vi "OverlayBitmapCenter.vi"(7 "GroupName":string, 8 "error in":errorcluster, 9 "Bitmap":u32[][](array[colorbox]), 10 "Center":T1, 11 "Image Reference In":T2) -> (0 "error out":errorcluster, 3 "Image Reference Out":T2)   [LabVIEW 2020, in "OpenLvVision_Overlays.lvlib"]
doc: "Overlays an bitmap on top of an image."
uses:
  OpenLvVision_Overlays.lvlib
  <vilib>/OpenLvVision/OpenLvVision_Image/Management/TypeDef/OLV Image.ctl
  TypeDefs/PointI32.ctl
  <vilib>/OpenLvVision/OpenLvVision_Image/Management/OLV Management.lvlib
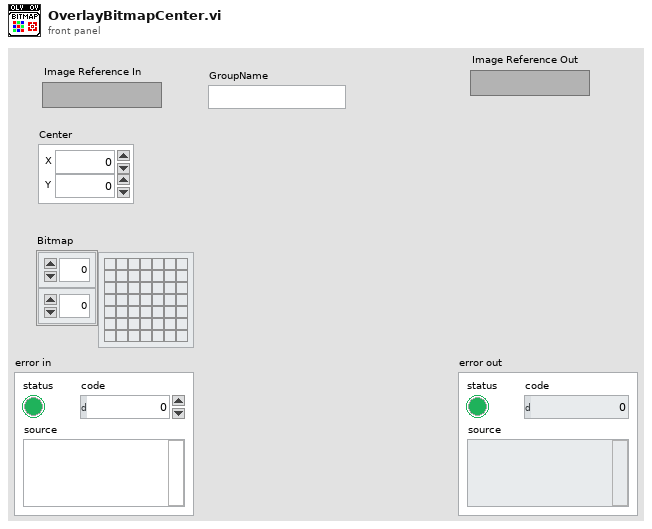
[diagram p1: front panel]
types:
  T1 = typedef "OpenLvVision_Overlays.lvlib/PointI32.ctl" = cluster{"X":i32, "Y":i32}
  T2 = typedef "OLV OpenLvVision_Image.lvlib/OLV Management.lvlib/OLV Image.ctl" = refnum<image>
  T3 = typedef "IMAQ Image.ctl" = refnum<image>
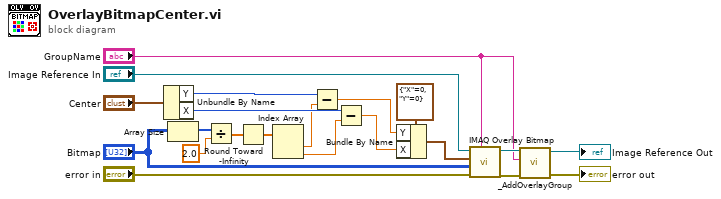
[diagram p0: block diagram]
diagram:
  n1 = Unbundle By Name("Center") -> ("Y"=w15:i32, "X"=w14:i32)
  n2 = Array Size(array="Bitmap") -> (size(s)=w18:i32[])
  n3 = Divide(x=w18, y=2.0) -> (x/y=w7:dbl[])
  n4 = Round Toward -Infinity(1:w7) -> (0:w6:dbl[])
  n5 = Index Array(array=w6) -> (element #1=w13:dbl, element #2=w12:dbl)  [unwired: 2 in]
  n6 = Subtract(x=w15, y=w13) -> (x-y=w10:dbl)
  n7 = Subtract(x=w14, y=w12) -> (x-y=w9:dbl)
  n8 = Bundle By Name(cluster=T1 {"X"=0, "Y"=0} ("Center"), "Y"=w10, "X"=w9) -> (w8:T1)
  n9 = call "IMAQ Overlay Bitmap"("Group"="GroupName", "error in (no error)"="error in", "Bitmap"="Bitmap", "Top Left Point"=w8, "Image"="Image Reference In") -> ("error out"=w4:errorcluster, "Image Out"=w5:T3)  [unwired: 5 in]
  n10 = call "_AddOverlayGroup.vi"("error in"=w4, "GroupName"="GroupName", "Image Reference In"=w5) -> ("error out"=→"error out":errorcluster, "Image Reference Out"=→"Image Reference Out":T2)  [unwired: 7 in]
